vi "MQTT Data - Encode U16.vi"(4 "U16":u16, 5 "remaining data in":u8[](array[numeric])) -> (2 "remaining data out":u8[](array[numeric]))   [LabVIEW 2019, in "KoRE-MQTT.lvlib"]
doc: "Copyright (c) 2025 KoRElibs.com\nSPDX-License-Identifier: EUPL-1.2\n\nThis VI is licensed under the European Union Public License (EUPL) Version 1.2. You may use this VI unmodified in proprietary works. If you distribute a modified version of this file, the modified file must be released under the EUPL-1.2. Full license: https://joinup.ec.europa.eu/asset/eupl/eupl/1.2/"
uses:
  KoRE-MQTT.lvlib
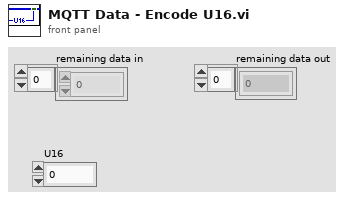
[diagram p1: front panel]
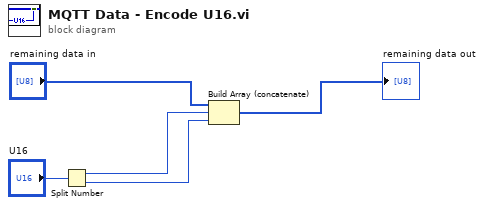
[diagram p0: block diagram]
diagram:
  n1 = Split Number(x="U16") -> (hi(x)=w3:u8, lo(x)=w2:u8)
  n2 = Build Array (concatenate)("remaining data in", w3, w2) -> (→"remaining data out":u8[])
